vi "Parallel Index VIs.vi"(7 "Queue in":refnum<queue>, 8 "error in (no error)":errorcluster, 9 "Parallel Instances (8)":i32=8, 10 "Node Progress ref":refnum<vi>, 11 "Example Files":path[](array[path])) -> (0 "error out":errorcluster, 2 "Indexed":set{string}(c389), 3 "File Data Array":T1[](array[typedef]))   [LabVIEW 2020]
uses:
  DBMap/DBMap.lvclass
  DBSet/DBSet.lvclass
  Indexer Action.ctl
  File Metadata.ctl
  Node.ctl
  Source to Sink Array.ctl
  File Data.ctl
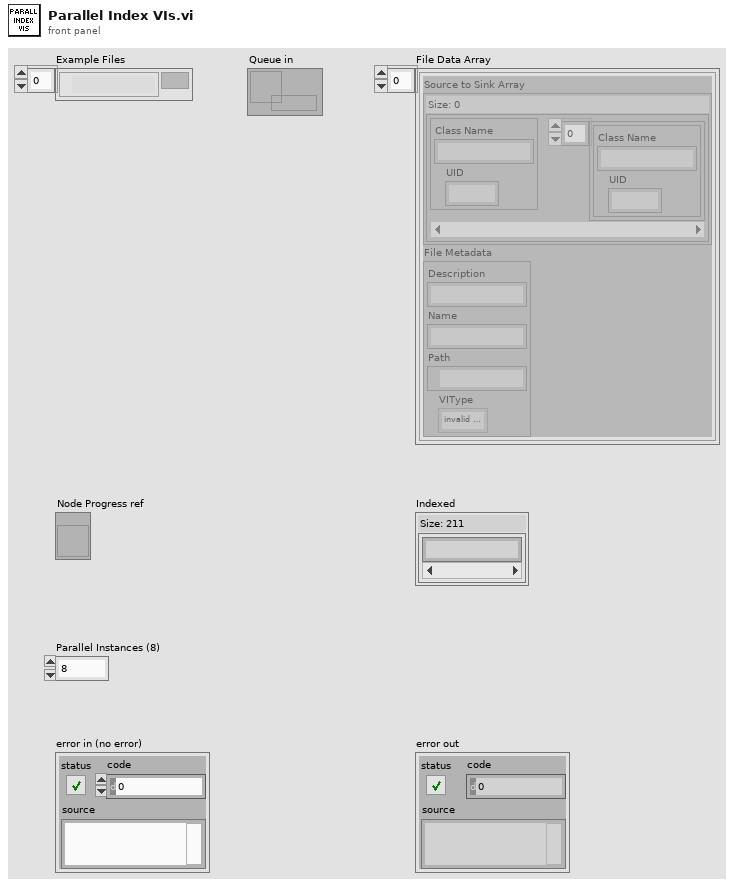
[diagram p1: front panel]
types:
  T1 = typedef "File Data.ctl" = cluster{"Source to Sink Array":T2, "File Metadata":T4}
  T2 = typedef "Source to Sink Array.ctl" = map{T3, T3[]}
  T3 = typedef "Node.ctl" = cluster{"Class Name":string, "UID":i32}
  T4 = typedef "File Metadata.ctl" = cluster{"Description":string, "Name":string, "Path":path, "VIType":enum32{"invalid VI type", "Standard VI", "Control VI", "Global VI", "Polymorphic VI", "Configuration VI", "SubSystem", "Facade VI", "Method VI", "Statechart Diagram VI"}}
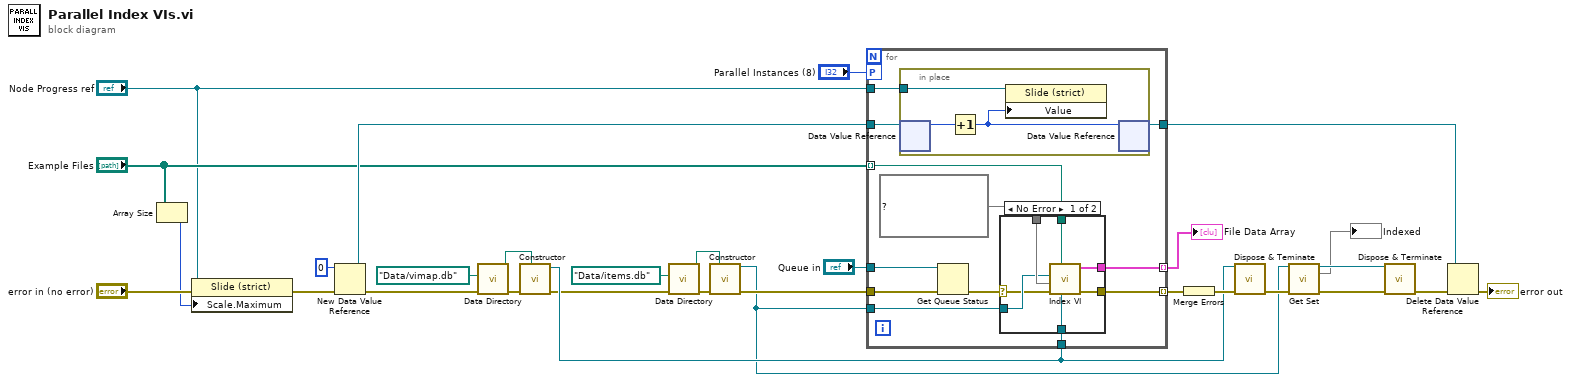
[diagram p0: block diagram]
diagram:
  n1 = Array Size(array="Example Files") -> (size(s)=w15:i32)
  n2 = property on="Property Node" class="Slide (strict)"(reference="Node Progress ref", error in="error in (no error)", "Scale.Maximum"=w15) -> (error out=w16:errorcluster)  [unwired: 1 out]
  n3 = New Data Value Reference(data value=u64 0, error in=w16) -> (data value reference=w29:refnum<data-value>, error out=w8:errorcluster)
  n4 = call "Data Directory.vi"("error in (no error)"=w8, "Subdirectory"=path "Data/vimap.db" ("name or relative path")) -> ("error out"=w7:errorcluster, "Data directory"=w6:path)  [unwired: 8 in]
  n5 = call "Constructor.vi"("SQLite DB Path"=w6, "error in (no error)"=w7) -> ("error out"=w3:errorcluster, "DBMap out"=w24:refnum<class "DBMap.lvclass">)  [unwired: 8 in]
  n6 = call "Data Directory.vi"("error in (no error)"=w3, "Subdirectory"=path "Data/items.db" ("name or relative path")) -> ("error out"=w4:errorcluster, "Data directory"=w2:path)  [unwired: 8 in]
  n7 = call "Constructor.vi"("SQLite DB Path"=w2, "error in (no error)"=w4) -> ("DBSet out"=w22:refnum<class "DBSet.lvclass">, "error out"=w23:errorcluster)  [unwired: 12 in]
  n8 = for {
    tunnel: "Example Files" -> [w41] mode=indexing
    tunnel: [w42] -> w1 mode=indexing
    tunnel: w29 -> [w40]
    tunnel: [w39] -> w28
    tunnel: w22 -> [w38]
    tunnel: w24 -> [w37]
    workers-P: "Parallel Instances (8)" -> [_]
    tunnel: w23 -> [w34]
    tunnel: [w36] -> w27 mode=indexing
    tunnel: "Queue in" -> [w35]
    tunnel: "Node Progress ref" -> [w31]
    n9 = in-place {
      in-place-border: w31 -> [w51]
      n10 = in-place-dvr #1(w40) -> (w52:u64)  [unwired: 1 out]
      n11 = Increment(x=w52) -> (x+1=w50:u64)
      n12 = property class="Slide (strict)"(reference=w51, "Value"=w50) -> ()  [unwired: 1 in, 2 out]
      n13 = in-place-dvr #1(w50) -> (w39:refnum<data-value>)  [unwired: 1 out]
    }
    n14 = Get Queue Status(queue=w35, error in (no error)=w34) -> (error out=w32:errorcluster)  [unwired: 1 in, 7 out]
    n15 = case shown="No Error" w32 {
      selector: w32 -> [w43 _]
      tunnel: set{string} {"ControlTerminal", "OverridableParameterTerminal", "ParameterTerminal", "Terminal"} ("Set") -> [w49 _]
      tunnel: [w48 _] -> w42
      tunnel: w41 -> [w47 _]
      tunnel: w38 -> [w46 _]
      tunnel: [w44 _] -> w36
      tunnel: w37 -> [w45 _]
      frame No Error {
        n16 = call "Index VI.vi"("DBMap"=w45, "VI to analyze"=w47, "error in (no error)"=w43, "Valid Terminals Set"=w49, "AtomicSet"=w46) -> ("error out"=w44:errorcluster, "File Data"=w48:T1)  [unwired: 5 in]
      }
      frame Error {
      }
    }
  }
  "File Data Array" <- w1
  n17 = Merge Errors(w27) -> (w26:errorcluster)
  n18 = call-dynamic "Dispose & Teminate.vi"("DBMap in"=w24, "error in (no error)"=w26) -> ("error out"=w25:errorcluster)  [unwired: 12 in, 1 out]
  n19 = call "Get Set.vi"("DBSet in"=w22, "error in (no error)"=w25) -> ("DBSet out"=w19:refnum<class "DBSet.lvclass">, "Set"=→"Indexed":set{string}, "error out"=w21:errorcluster)  [unwired: 11 in]
  n20 = call-dynamic "Dispose & Terminate.vi"("DBSet in"=w19, "error in (no error)"=w21) -> ("error out"=w20:errorcluster)  [unwired: 12 in, 1 out]
  n21 = Delete Data Value Reference(data value reference=w28, error in=w20) -> (error out=→"error out":errorcluster)  [unwired: 1 out]
